vi "Create Single AI.vi"(7 "section":string="Motor", 8 "error in (no error)":errorcluster, 9 "AI_Channel":string(combo)="Speed_AI_Channel", 10 "Modbus_Master.lvclass":refnum<class "Modbus_Master.lvclass">, 11 "Path In":path) -> (0 "error out":errorcluster, 2 "AnalogInput.lvclass":refnum<class "AnalogInput.lvclass">, 3 "Path Out":path)   [LabVIEW 2021]
uses:
  AnalogInput/AnalogInput.lvclass
  Modbus_Master/Modbus_Master.lvclass
  Modbus_AI/Modbus_AI.lvclass
  C:/Users/lincoln.lucio/Documents/Lincoln/Documentos Pessoais/meus docs/Projetos pessoais/Projeto Sciranda/projeto_versioned/sciranda/AnalogInput/AnalogInput.lvclass
  Modbus_AI/Modbus_AI.lvclass/Modbus_AI.ctl
  DAQNavi_AI.lvclass/DAQNavi_AI.lvclass
  DAQNavi_AI.lvclass/DAQNavi_AI.lvclass/DAQNavi_AI.ctl
  Modbus_AI/Accessor VIs/Write Modbus_Master.lvclass.vi
  Modbus_AI/Accessor VIs/Write Register Address.vi
  Modbus_AI/Accessor VIs/Write Is Signed (I16)_.vi
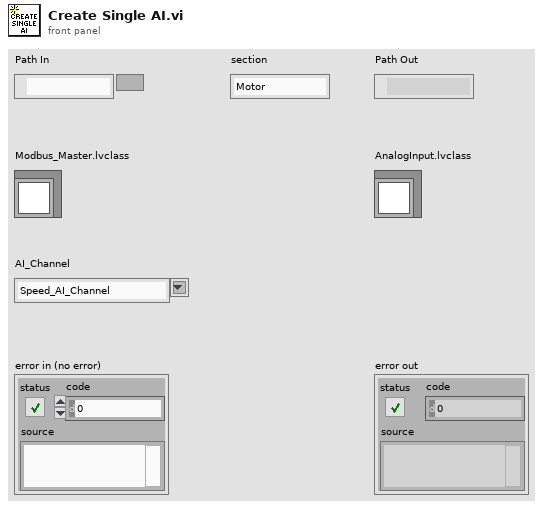
[diagram p1: front panel]
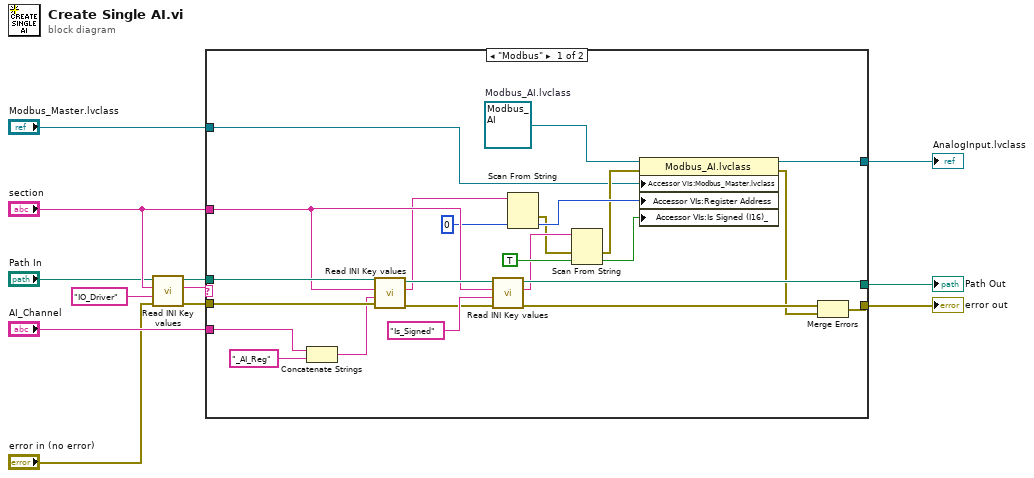
[diagram p0: block diagram]
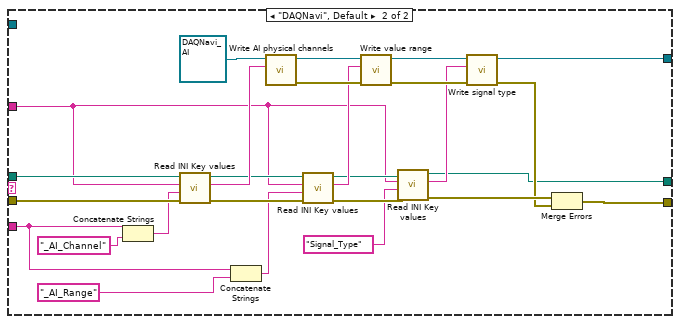
[diagram p2: hidden frame]
diagram:
  n1 = call "Read INI Key values.vi"("error in (no error)"="error in (no error)", "key"="IO_Driver", "section"="section", "Path In"="Path In") -> ("error out"=w4:errorcluster, "value"=w9:string, "Path Out"=w6:path)  [unwired: 5 in]
  n2 = case shown="\"Modbus\"" w9 {
    tunnel: w6 -> [w36 w61]
    tunnel: "AI_Channel" -> [w14 w37]
    tunnel: "section" -> [w28 w50]
    tunnel: w4 -> [w35 w48]
    tunnel: [w17 w45] -> w11
    tunnel: [w26 w44] -> w2
    tunnel: [w30 w43] -> w10
    tunnel: "Modbus_Master.lvclass" -> [w13 _]
    frame "Modbus" {
      w27 = refnum<class "Modbus_AI.lvclass"> refnum  # Modbus_AI.lvclass
      n3 = Concatenate Strings(w14, "_AI_Reg" ("key")) -> (w15:string)
      n4 = call "Read INI Key values.vi"("error in (no error)"=w35, "key"=w15, "section"=w28, "Path In"=w36) -> ("error out"=w31:errorcluster, "value"=w24:string, "Path Out"=w32:path)  [unwired: 5 in]
      n5 = call "Read INI Key values.vi"("error in (no error)"=w31, "key"="Is_Signed", "section"=w28, "Path In"=w32) -> ("error out"=w29:errorcluster, "value"=w21:string, "Path Out"=w30:path)  [unwired: 5 in]
      n6 = Scan From String(input string=w24, default 1=u16 0 ("Register Address")) -> (error out=w19:errorcluster, output 1=w23:u16)  [unwired: 3 in, 2 out]
      n7 = Scan From String(input string=w21, error in=w19, default 1=TRUE ("Is Signed (I16)_")) -> (error out=w18:errorcluster, output 1=w20:bool)  [unwired: 2 in, 2 out]
      n8 = property class="Modbus_AI.lvclass"(reference=w27, error in=w18, "Accessor VIs:Modbus_Master.lvclass"=w13, "Accessor VIs:Register Address"=w23, "Accessor VIs:Is Signed (I16)_"=w20) -> (reference out=w26:refnum<class "Modbus_AI.lvclass">, error out=w16:errorcluster)
      n9 = Merge Errors(w29, w16) -> (w17:errorcluster)
    }
    frame "DAQNavi", Default {
      n10 = Concatenate Strings(w37, "_AI_Channel" ("AI_Channel")) -> (w40:string)
      n11 = call "Read INI Key values.vi"("error in (no error)"=w48, "key"=w40, "section"=w50, "Path In"=w61) -> ("error out"=w58:errorcluster, "value"=w60:string, "Path Out"=w59:path)  [unwired: 5 in]
      n12 = Concatenate Strings(w37, "_AI_Range" ("AI_Range")) -> (w39:string)
      n13 = call "Write AI physical channels.vi"("physical channels"=w60, "DAQNavi_AI in"=refnum<class "DAQNavi_AI.lvclass"> refnum ("DAQNavi_AI.lvclass")) -> ("error out"=w56:errorcluster, "DAQNavi_AI out"=w57:refnum<class "DAQNavi_AI.lvclass">)  [unwired: 8 in]
      n14 = call "Read INI Key values.vi"("error in (no error)"=w58, "key"=w39, "section"=w50, "Path In"=w59) -> ("error out"=w51:errorcluster, "value"=w53:string, "Path Out"=w52:path)  [unwired: 5 in]
      n15 = call "Write value range.vi"("error in (no error)"=w56, "value range"=w53, "DAQNavi_AI in"=w57) -> ("error out"=w54:errorcluster, "DAQNavi_AI out"=w55:refnum<class "DAQNavi_AI.lvclass">)  [unwired: 7 in]
      n16 = call "Read INI Key values.vi"("error in (no error)"=w51, "key"="Signal_Type" ("Signal_Type"), "section"=w50, "Path In"=w52) -> ("error out"=w47:errorcluster, "value"=w49:string, "Path Out"=w43:path)  [unwired: 5 in]
      n17 = call "Write signal type.vi"("error in (no error)"=w54, "signal type"=w49, "DAQNavi_AI in"=w55) -> ("error out"=w46:errorcluster, "DAQNavi_AI out"=w44:refnum<class "DAQNavi_AI.lvclass">)  [unwired: 7 in]
      n18 = Merge Errors(w47, w46) -> (w45:errorcluster)
    }
  }
  "error out" <- w11
  "Path Out" <- w10
  "AnalogInput.lvclass" <- w2
